vi "HostMem ReleasePointer.vi"(8 "error in (no error)":errorcluster, 11 "PointerData":T1) -> (0 "error out":errorcluster)   [LabVIEW 2020, in "OpenLvVision_OpenCv.lvlib" / "Cuda.lvlib" / "HostMem.lvclass"]
doc: "Manually releases a pinned memory handle previously generated by the Get Pointer VI."
uses:
  HostMem.lvclass
  TypeDef/HostMem PointerData.ctl
  TypeDef/cvType.ctl
  OpenLvVision_OpenCv.lvlib
  <vilib>/Utility/error.llb/Error Cluster From Error Code.vi
  <vilib>/ErrorRing/Error Ring.xnode
  Dlls/OlvOpenCvWrapper.dll
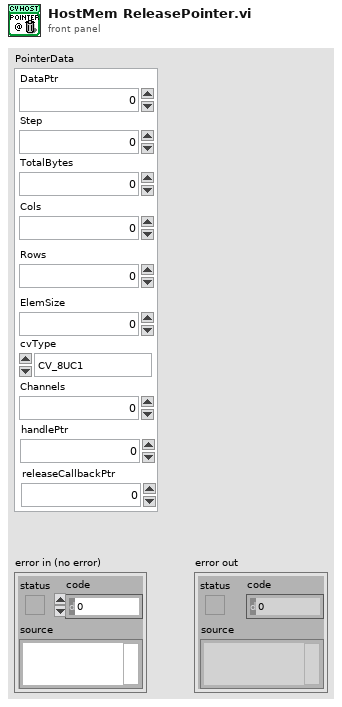
[diagram p1: front panel]
types:
  T1 = typedef "OpenLvVision_OpenCv.lvlib/HostMem PointerData.ctl" = cluster{"DataPtr":u64, "Step":i64, "TotalBytes":u64, "Cols":i32, "Rows":i32, "ElemSize":i32, "cvType":T2, "Channels":i32, "handlePtr":u64, "releaseCallbackPtr":u64}
  T2 = typedef "OpenLvVision_OpenCv.lvlib/cvType.ctl" = enum32{"CV_8UC1", "CV_8SC1", "CV_16UC1", "CV_16SC1", "CV_32SC1", "CV_32FC1", "CV_64FC1", "CV_16FC1", "CV_8UC2", "CV_8SC2", "CV_16UC2", "CV_16SC2", "CV_32SC2", "CV_32FC2", "CV_64FC2", "CV_16FC2", "CV_8UC3", "CV_8SC3", "CV_16UC3", "CV_16SC3", "CV_32SC3", "CV_32FC3", "CV_64FC3", "CV_16FC3", "CV_8UC4", "CV_8SC4", "CV_16UC4", "CV_16SC4", "CV_32SC4", "CV_32FC4", "CV_64FC4", "CV_16FC4"}
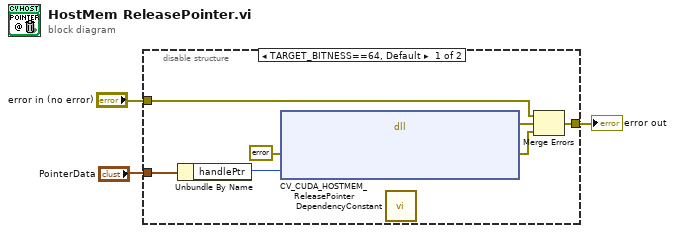
[diagram p0: block diagram]
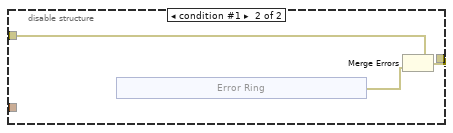
[diagram p2: hidden frame]
diagram:
  n1 = disable-structure shown="TARGET_BITNESS==64, Default" {
    disable-tunnel: "error in (no error)" -> [w5 w12]
    disable-tunnel: [w4 w13] -> w2
    disable-tunnel: "PointerData" -> [w10 _]
    frame condition #0 (active) {
      n2 = Unbundle By Name(w10) -> ("handlePtr"=w6:u64)
      n3 = dll-call lib="C:/Users/lukas/Documents/OpenLvVision_OpenCv/SourceCode/LabView/OpenLvVision_OpenCv/Dlls/OlvOpenCvWrapper.dll" fn="CV_CUDA_HOSTMEM_ReleasePointer"("Error"=errorcluster {"status"=FALSE, "code"=0, "source"=""} ("error out"), "handle"=w6) -> (error out=w9:errorcluster, "Error"=w8:errorcluster)  [unwired: 5 in, 1 out]
      n4 = call "DependencyConstant.vi"() -> ()  [unwired: 12 in]
      n5 = Merge Errors(w5, w9, w8) -> (w4:errorcluster)
    }
    frame condition #1 {
      n6 = xnode "Error Ring"() -> ("error out"=w11:errorcluster)
      n7 = Merge Errors(w12, w11) -> (w13:errorcluster)
    }
  }
  "error out" <- w2
